vi "WeightCalculator.vi"(1 "Cp":dbl, 2 "vC":dbl, 3 "Lc":dbl) -> (0 "W":dbl)   [LabVIEW 2024]
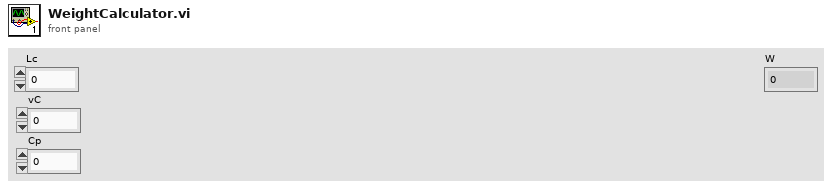
[diagram p1: front panel]
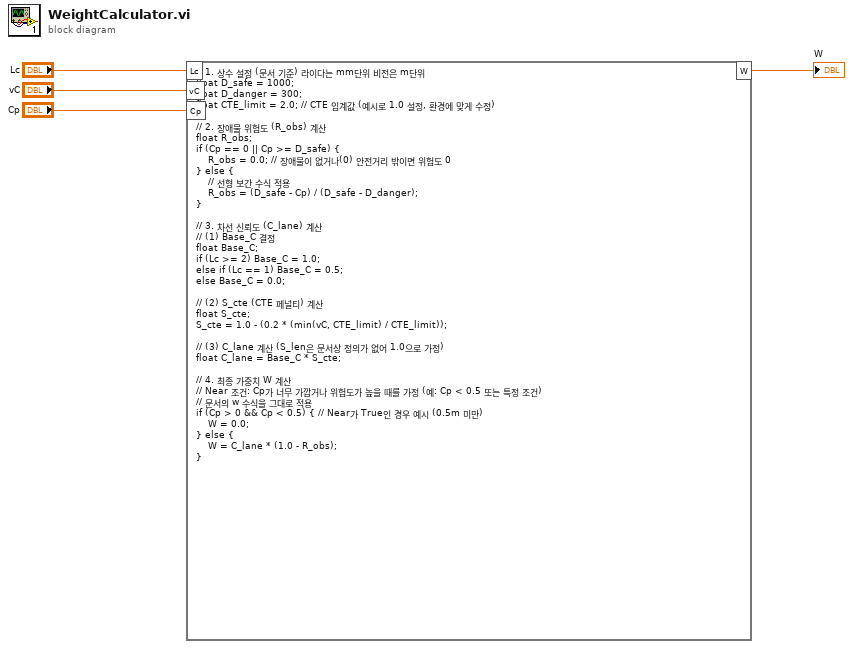
[diagram p0: block diagram]
diagram:
  n1 = formula code="// 1. 상수 설정 (문서 기준) 라이다는 mm단위 비전은 m단위\nfloat D_safe = 1000;\nfloat D_danger = 300;\nfloat CTE_limit = 2.0; // CTE 임계값 (예시로 1.0 설정, 환경에 맞게 수정)\n\n// 2. 장애물 위험도 (R_obs) 계산\nfloat R_obs;\nif (Cp == 0 || Cp >= D_safe) { \n    R_obs = 0.0; // 장애물이 없거나(0) 안전거리 밖이면 위험도 0\n} else {\n    // 선형 보간 수식 적용\n    R_obs = (D_safe - Cp) / (D_safe - D_danger);\n}\n\n// 3. 차선 신뢰도 (C_lane) 계산\n// (1) Base_C 결정\nfloat Base_C;\nif (Lc >= 2) Base_C = 1.0;\nelse if (Lc == 1) Base_C = 0.5;\nelse Base_C = 0.0;\n\n// (2) S_cte (CTE 페널티) 계산\nfloat S_cte;\nS_cte = 1.0 - (0.2 * (min(vC, CTE_limit) / CTE_limit));\n\n// (3) C_lane 계산 (S_len은 문서상 정의가 없어 1.0으로 가정)\nfloat C_lane = Base_C * S_cte;\n\n// 4. 최종 가중치 W 계산\n// Near 조건: Cp가 너무 가깝거나 위험도가 높을 때를 가정 (예: Cp < 0.5 또는 특정 조건)\n// 문서의 w 수식을 그대로 적용\nif (Cp > 0 && Cp < 0.5) { // Near가 True인 경우 예시 (0.5m 미만)\n    W = 0.0;\n} else {\n    W = C_lane * (1.0 - R_obs);\n}"("Lc"="Lc", "vC"="vC", "Cp"="Cp") -> ("W"=→"W":dbl)
